vi "SC Reopen Project.vi"(8 "error in (no error)":errorcluster, 9 "project path":path, 10 "new file":string) -> (0 "error out":errorcluster)   [LabVIEW 2023]
doc: "Opens the project again after systemcore-deploy changed its files: the same .lvproj when it still exists, otherwise the file systemcore-deploy named in its OPEN line (the new version's .lvproj; none if it has no project). Run it after any dialog has closed."
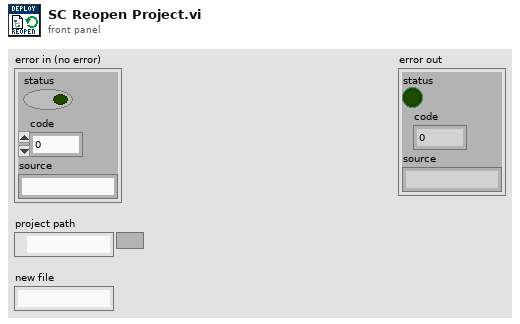
[diagram p1: front panel]
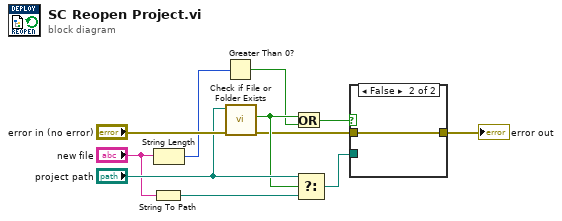
[diagram p0: block diagram]
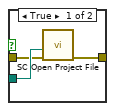
[diagram p2: hidden frame]
diagram:
  n1 = String To Path(string="new file") -> (path=w9:path)
  n2 = String Length(string="new file") -> (length=w7:i32)
  n3 = Greater Than 0?(x=w7) -> (x > 0?=w5:bool)
  n4 = call <vilib>:"Check if File or Folder Exists.vi"("error in (no error)"="error in (no error)", "path"="project path") -> ("error out"=w3:errorcluster, "file or folder exists?"=w6:bool)  [unwired: 7 in, 1 out]
  n5 = Or(x=w6, y=w5) -> (x .or. y?=w1:bool)
  n6 = Select(t="project path", s=w6, f=w9) -> (s? t:f=w4:path)
  n7 = case shown="False" w1 {
    tunnel: w4 -> [w14 _]
    tunnel: w3 -> [w13 w15]
    tunnel: [w12 w15] -> w2
    frame True {
      n8 = call "SC Open Project File.vi"("error in (no error)"=w13, "path"=w14) -> ("error out"=w12:errorcluster)  [unwired: 9 in]
    }
    frame False {
    }
  }
  "error out" <- w2
